vi "SimulatorOscilloscope.vi"() -> ()   [LabVIEW 2014]
uses:
  SimulatorGlobalOscilloscope.vi
panel:
  out "ChkSum Error":bool
  out "Sync Error":bool
  out "Timeout Error":bool
  in  "SimulatorOscilloscope":T1(tab)=enum."Oscilloscope"
  in  "Voltage Reference":dbl caption="V"
  in  "ChkSum":enum16{"ZERO16", "LRC8", "CRC16-CCITT"}(ring)
  in  "Serial Port":T2(ring)
  in  "Baud Rate":u32=9600
  in  "timeout [ms]":u32=10000
  in  "SW":u8
  in  "BTN0":bool
  in  "BTN1":bool
  in  "BTN2":bool
  in  "BTN3":bool
  out "FreqSelect":bool
  out "AmplSelect":bool
  out "ShapeSelect":bool=TRUE
  out "Shape1Index":u8
  out "AmplIndex":u8
  out "FreqIndex":u8
  out "Frequency":string="   0,0Hz"
  out "Amplitude":string="   0,00 V"
  out "Shape":string="Const"
  in  "Number of Packets shown":i16=2
  in  "SEND Button":bool
  in  "Record Length":u16=500
  in  "Sample Rate":u16=10000
  out "Oscilloskop":u8[](graph)
  out "XY Graph":cluster{u32[], dbl[]}(graph)
  in  "Start":bool
  out "Raw Packet":string
  out "Raw":string
  # "Received raw data (in hex)"
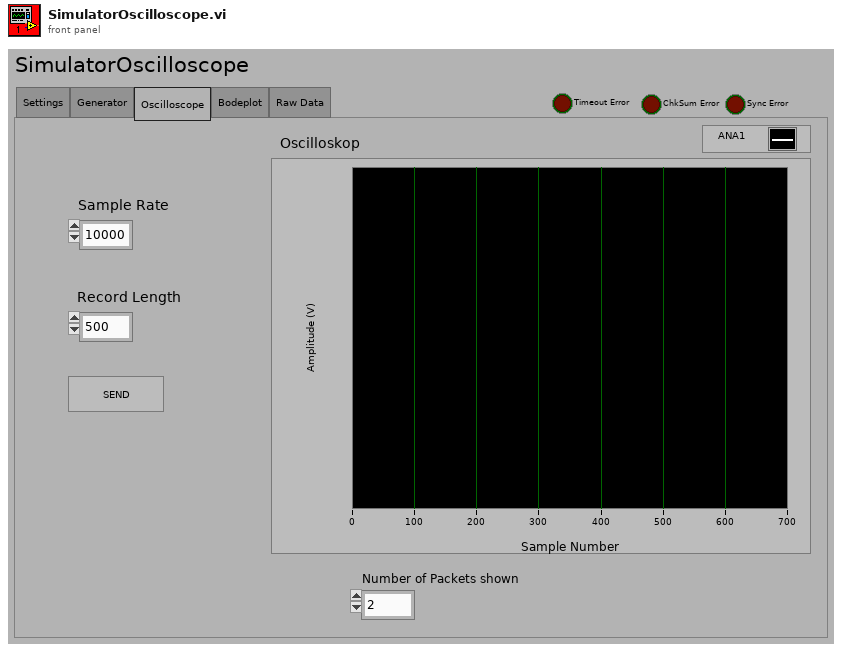
[diagram p1: front panel]
types:
  T1 = enum32{"Settings", "Generator", "Oscilloscope", "Bodeplot", "Raw Data"}
  T2 = enum16{"COM1", "COM2", "COM3", "COM4", "COM5", "COM6", "COM7", "COM8", "COM9", "COM10", "COM11", "COM12", "COM13", "COM14", "COM15", "COM16", "COM17", "COM18", "COM19", "COM20", "COM21", "COM22", "COM23", "COM24", "COM25", "COM26", "COM27", "COM28", "COM29", "COM30"}
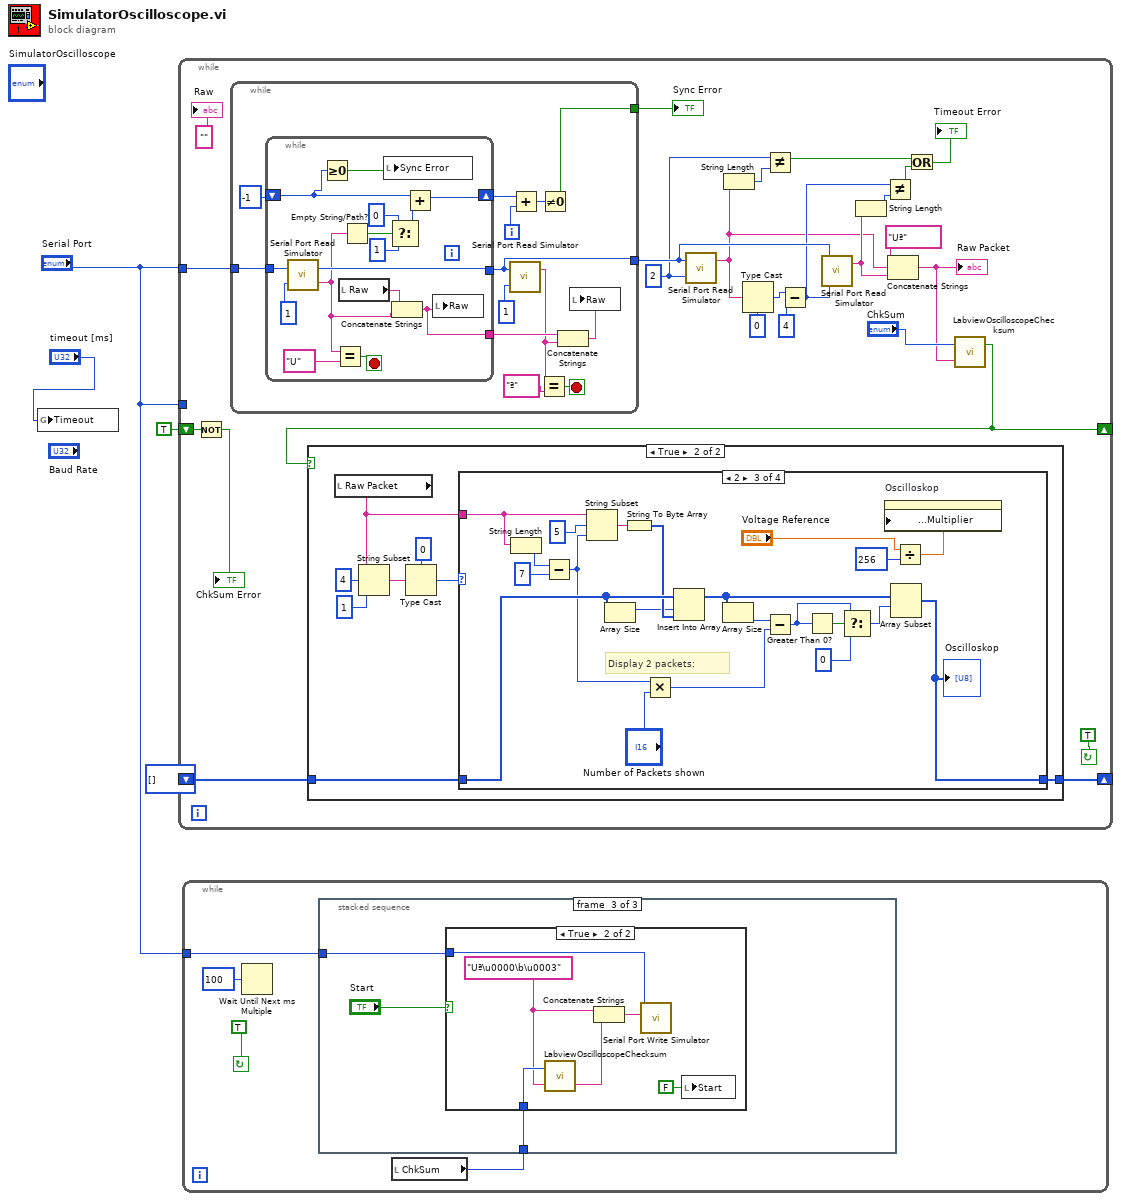
[diagram p0: block diagram]
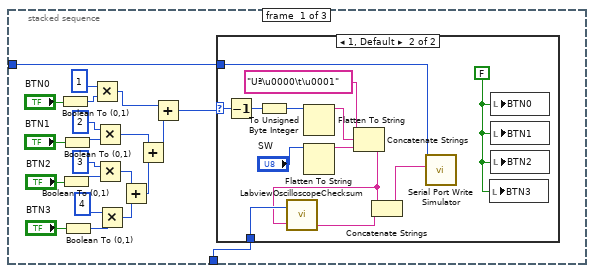
[diagram p2: hidden frame]
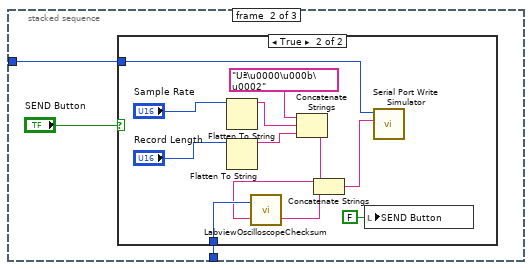
[diagram p4: hidden frame]
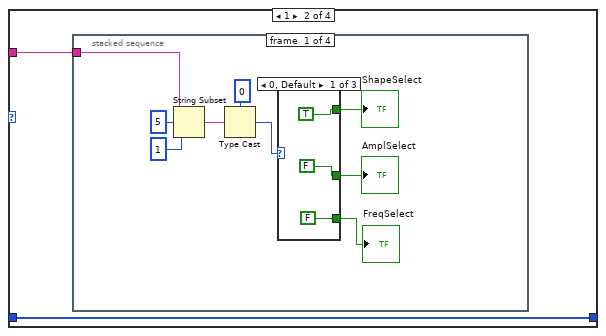
[diagram p9: hidden frame]
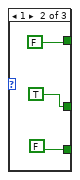
[diagram p10: hidden frame]
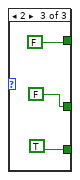
[diagram p11: hidden frame]
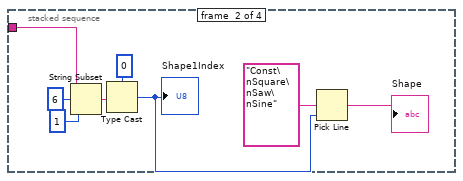
[diagram p12: hidden frame]
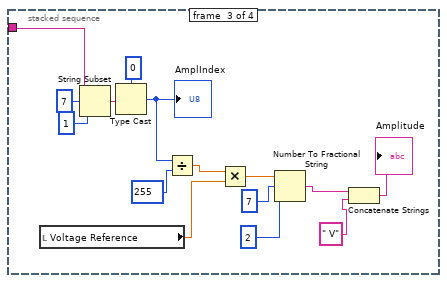
[diagram p13: hidden frame]
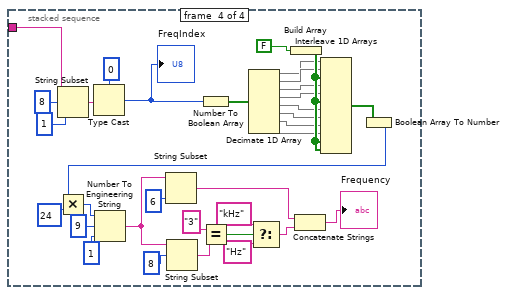
[diagram p14: hidden frame]
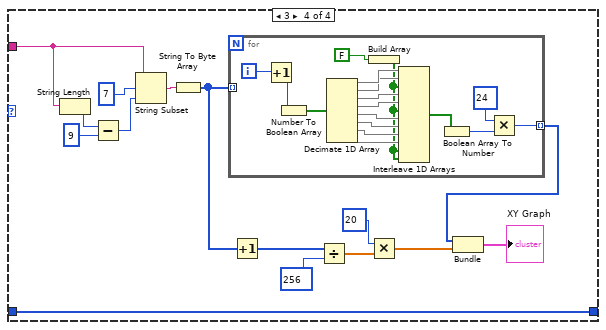
[diagram p15: hidden frame]
diagram:
  n1 = global write "SimulatorGlobalOscilloscope.vi" "Timeout"("timeout [ms]") -> ()
  n2 = while {
    shift-right: [w29] -> _
    shift-left: u8[] [] -> [w28]
    tunnel: "Serial Port" -> [w21]
    shift-right: [w7] -> _
    shift-left: TRUE -> [w6]
    tunnel: "Serial Port" -> [_]
    stop <- TRUE continue-if-true
    w15 = 2
    n3 = Not(x=w6) -> (.not. x?=→"ChkSum Error":bool)
    n4 = while {
      tunnel: w21 -> [w182]
      tunnel: [w177] -> w24
      tunnel: [w178] -> w20
      i -> [w173]
      stop <- w181 stop-if-true
      n5 = while {
        tunnel: w182 -> [w193]
        tunnel: [w193] -> w177
        tunnel: [w183] -> w180
        shift-right: [w185] -> w172
        shift-left: -1 -> [w187]
        stop <- w195 stop-if-true
        n6 = call "Serial Port Read Simulator.vi"("requested byte count"=1, "port number"=w193) -> ("string read"=w184:string)  [unwired: 1 out]
        n7 = Greater Or Equal To 0?(x=w187) -> (x >= 0?=w186:bool)
        n8 = Equal?(x=w184, y="U") -> (x = y?=w195:bool)
        n9 = local read "Raw"() -> (w192:string)
        n10 = Empty String/Path?(string/path=w184) -> (empty?=w188:bool)
        n11 = local write "Sync Error"(w186) -> ()
        n12 = Select(t=0, s=w188, f=1) -> (s? t:f=w189:i32)
        n13 = Concatenate Strings(w192, w184) -> (w183:string)
        n14 = Add(x=w187, y=w189) -> (x+y=w185:i32)
        n15 = local write "Raw"(w183) -> ()
      }
      n16 = call "Serial Port Read Simulator.vi"("requested byte count"=1, "port number"=w177) -> ("string read"=w171:string)  [unwired: 1 out]
      n17 = Add(x=w172, y=w173) -> (x+y=w179:i32)
      n18 = Equal?(x=w171, y="ª") -> (x = y?=w181:bool)
      n19 = Not Equal To 0?(x=w179) -> (x != 0?=w178:bool)
      n20 = Concatenate Strings(w180, w171) -> (w175:string)
      n21 = local write "Raw"(w175) -> ()
    }
    "Sync Error" <- w20
    n22 = call "Serial Port Read Simulator.vi"("requested byte count"=w15, "port number"=w24) -> ("string read"=w11:string)  [unwired: 1 out]
    n23 = String Length(string=w11) -> (length=w18:i32)
    n24 = Type Cast(type=i16 0, x=w11) -> (*(type *) &x=w25:i16)
    n25 = Not Equal?(x=w15, y=w18) -> (x != y?=w16:bool)
    n26 = Subtract(x=w25, y=i16 4) -> (x-y=w14:i16)
    n27 = call "Serial Port Read Simulator.vi"("requested byte count"=w14, "port number"=w24) -> ("string read"=w12:string)  [unwired: 1 out]
    n28 = String Length(string=w12) -> (length=w19:i32)
    n29 = Not Equal?(x=w14, y=w19) -> (x != y?=w17:bool)
    n30 = Concatenate Strings("Uª", w11, w12) -> (w8:string)
    "Raw Packet" <- w8
    n31 = Or(x=w16, y=w17) -> (x .or. y?=→"Timeout Error":bool)
    n32 = call "LabviewOscilloscopeChecksum.vi"("DATA PACKET"=w8, "ChkSumType"="ChkSum") -> ("Checked"=w7:bool)  [unwired: 1 out]
    n33 = case shown="True" w7 {
      tunnel: [w30 w38] -> w29
      tunnel: w28 -> [w30 w37]
      frame False {
      }
      frame True {
        n34 = local read "Raw Packet"() -> (w33:string)
        n35 = String Subset(string=w33, offset (0)=4, length (rest)=1 ("length (rest)")) -> (substring=w36:string)
        n36 = Type Cast(type=u8 0, x=w36) -> (*(type *) &x=w32:u8)
        n37 = case shown="2" w32 {
          tunnel: w33 -> [_ w41 w118 w147]
          tunnel: [w39 w40 w123 w138] -> w38
          tunnel: w37 -> [w39 w40 w131 w138]
          frame 0, Default {
          }
          frame 1 {
            n38 = stacked-sequence {
              tunnel: w41 -> [w48 w63 w78 w112]
              frame #0 {
                n39 = String Subset(string=w48, offset (0)=5, length (rest)=1 ("length (rest)")) -> (substring=w47:string)
                n40 = Type Cast(type=u8 0, x=w47) -> (*(type *) &x=w45:u8)
                n41 = case shown="0, Default" w45 {
                  tunnel: [TRUE FALSE FALSE] -> w44
                  tunnel: [FALSE TRUE FALSE] -> w43
                  tunnel: [FALSE FALSE TRUE] -> w42
                  frame 0, Default {
                  }
                  frame 1 {
                  }
                  frame 2 {
                  }
                }
                "ShapeSelect" <- w44
                "AmplSelect" <- w43
                "FreqSelect" <- w42
              }
              frame #1 {
                n42 = String Subset(string=w63, offset (0)=6, length (rest)=1 ("length (rest)")) -> (substring=w65:string)
                n43 = Type Cast(type=u8 0, x=w65) -> (*(type *) &x=w61:u8)
                "Shape1Index" <- w61
                n44 = Pick Line(multi-line string="Const\nSquare\nSaw\nSine", line index=w61) -> (output string=→"Shape":string)  [unwired: 1 in]
              }
              frame #2 {
                n45 = local read "Voltage Reference"() -> (w68:dbl)
                n46 = String Subset(string=w78, offset (0)=7, length (rest)=1 ("length (rest)")) -> (substring=w81:string)
                n47 = Type Cast(type=u8 0, x=w81) -> (*(type *) &x=w77:u8)
                "AmplIndex" <- w77
                n48 = Divide(x=w77, y=255) -> (x/y=w75:dbl)
                n49 = Multiply(x=w75, y=w68) -> (x*y=w74:dbl)
                n50 = Number To Fractional String(number=w74, width (-)=7, precision (6)=2) -> (F-format string=w71:string)  [unwired: 1 in]
                n51 = Concatenate Strings(w71, " V") -> (→"Amplitude":string)
              }
              frame #3 {
                n52 = String Subset(string=w112, offset (0)=8, length (rest)=1 ("length (rest)")) -> (substring=w114:string)
                n53 = Type Cast(type=u8 0, x=w114) -> (*(type *) &x=w84:u8)
                "FreqIndex" <- w84
                n54 = Number To Boolean Array(number=w84) -> (Boolean array=w86:bool[])
                n55 = Decimate 1D Array(w86) -> (w87:bool[], w93:bool[], w88:bool[], w94:bool[], w89:bool[], w90:bool[], w91:bool[], w95:bool[])
                n56 = Build Array(FALSE) -> (w96:bool[])
                n57 = Interleave 1D Arrays(w87, w93, w96, w88, w94, w96, w89, w90, w91, w95, w96, w96) -> (w92:bool[])
                n58 = Boolean Array To Number(Boolean array=w92) -> (number=w97:u32)
                n59 = Multiply(x=w97, y=24) -> (x*y=w99:u32)
                n60 = Number To Engineering String(2:1, 3:9, 4:w99) -> (0:w104:string)  [unwired: 1 in]
                n61 = String Subset(string=w104, length (rest)=6) -> (substring=w111:string)  [unwired: 1 in]
                n62 = String Subset(string=w104, offset (0)=8) -> (substring=w109:string)  [unwired: 1 in]
                n63 = Equal?(x="3", y=w109) -> (x = y?=w107:bool)
                n64 = Select(t="kHz", s=w107, f="Hz") -> (s? t:f=w110:string)
                n65 = Concatenate Strings(w111, w110) -> (→"Frequency":string)
              }
            }
          }
          frame 2 {
            # "Display 2 packets:"
            n66 = String Length(string=w118) -> (length=w137:i32)
            n67 = Subtract(x=w137, y=7 ("length (rest)")) -> (x-y=w119:i32)
            n68 = String Subset(string=w118, offset (0)=5, length (rest)=w119) -> (substring=w134:string)
            n69 = Array Size(array=w131) -> (size(s)=w129:i32)
            n70 = String To Byte Array(string=w134) -> (unsigned byte array=w130:u8[])
            n71 = Multiply(x=w119, y="Number of Packets shown") -> (x*y=w121:i32)
            n72 = Insert Into Array(array=w131, index=w129, new element=w130) -> (w124:u8[])
            n73 = Array Size(array=w124) -> (size(s)=w126:i32)
            n74 = Subtract(x=w126, y=w121) -> (x-y=w127:i32)
            n75 = Greater Than 0?(x=w127) -> (x > 0?=w128:bool)
            n76 = Select(t=w127, s=w128, f=0) -> (s? t:f=w122:i32)
            n77 = Array Subset(array=w124, index=w122) -> (w123:u8[])  [unwired: 1 in]
            "Oscilloskop" <- w123
            n78 = Divide(x="Voltage Reference", y=u16 256) -> (x/y=w132:dbl)
            n79 = property on="Oscilloskop" class="WFGraph (strict)"("Y Scale.Offset and Multiplier:Multiplier"=w132) -> ()  [unwired: 2 in, 2 out]
          }
          frame 3 {
            n80 = String Length(string=w147) -> (length=w149:i32)
            n81 = Subtract(x=w149, y=9 ("length (rest)")) -> (x-y=w148:i32)
            n82 = String Subset(string=w147, offset (0)=7, length (rest)=w148) -> (substring=w152:string)
            n83 = String To Byte Array(string=w152) -> (unsigned byte array=w143:u8[])
            n84 = for {
              tunnel: [w155] -> w146 mode=indexing
              tunnel: w143 -> [_] mode=indexing
              i -> [w157]
              n85 = Increment(x=w157) -> (x+1=w156:i32)
              n86 = Number To Boolean Array(number=w156) -> (Boolean array=w168:bool[])
              n87 = Decimate 1D Array(w168) -> (w167:bool[], w161:bool[], w166:bool[], w160:bool[], w165:bool[], w164:bool[], w163:bool[], w159:bool[])
              n88 = Build Array(FALSE) -> (w158:bool[])
              n89 = Interleave 1D Arrays(w167, w161, w158, w166, w160, w158, w165, w164, w163, w159, w158, w158) -> (w162:bool[])
              n90 = Boolean Array To Number(Boolean array=w162) -> (number=w154:u32)
              n91 = Multiply(x=24, y=w154) -> (x*y=w155:u32)
            }
            n92 = Increment(x=w143) -> (x+1=w139:u8[])
            n93 = Divide(x=w139, y=256) -> (x/y=w142:dbl[])
            n94 = Multiply(x=20, y=w142) -> (x*y=w140:dbl[])
            n95 = Bundle(w146, w140) -> (→"XY Graph":cluster{u32[], dbl[]})  [unwired: 1 in]
          }
        }
      }
    }
    "Raw" <- ""
  }
  n96 = while {
    tunnel: "Serial Port" -> [w198]
    stop <- TRUE continue-if-true
    n97 = Wait Until Next ms Multiple(millisecond multiple=100) -> ()  [unwired: 1 out]
    n98 = local read "ChkSum"() -> (w197:enum16{"ZERO16", "LRC8", "CRC16-CCITT"})
    n99 = stacked-sequence {
      tunnel: w198 -> [w221 w236 w250]
      tunnel: w197 -> [w220 w235 w249]
      frame #0 {
        n100 = Boolean To (0,1)(Boolean="BTN0") -> (0, 1=w215:i16)
        n101 = Boolean To (0,1)(Boolean="BTN2") -> (0, 1=w211:i16)
        n102 = Boolean To (0,1)(Boolean="BTN1") -> (0, 1=w209:i16)
        n103 = Boolean To (0,1)(Boolean="BTN3") -> (0, 1=w213:i16)
        n104 = Multiply(x=u8 1, y=w215) -> (x*y=w207:i16)
        n105 = Multiply(x=u8 2, y=w209) -> (x*y=w205:i16)
        n106 = Multiply(x=u8 3, y=w211) -> (x*y=w203:i16)
        n107 = Multiply(x=u8 4, y=w213) -> (x*y=w204:i16)
        n108 = Add(x=w203, y=w204) -> (x+y=w202:i16)
        n109 = Add(x=w205, y=w202) -> (x+y=w206:i16)
        n110 = Add(x=w207, y=w206) -> (x+y=w201:i16)
        n111 = case shown="1, Default" w201 {
          selector: w201 -> [_ w230]
          tunnel: w221 -> [_ w224]
          tunnel: w220 -> [_ w228]
          frame 0 {
          }
          frame 1, Default {
            w231 = FALSE
            n112 = Decrement(x=w230) -> (x-1=w225:i16)
            n113 = To Unsigned Byte Integer(number=w225) -> (unsigned 8bit integer=w222:u8)
            n114 = Flatten To String(anything=w222) -> (data string=w229:string)  [unwired: 3 in, 2 out]
            n115 = Flatten To String(anything="SW") -> (data string=w232:string)  [unwired: 3 in, 2 out]
            n116 = Concatenate Strings("Uª\u0000\t\u0001", w229, w232) -> (w226:string)
            n117 = call "LabviewOscilloscopeChecksum.vi"("DATA PACKET"=w226, "ChkSumType"=w228) -> ("ChkSum"=w227:string)  [unwired: 1 out]
            n118 = Concatenate Strings(w226, w227) -> (w223:string)
            n119 = call "Serial Port Write Simulator.vi"("Port"=w224, "String"=w223) -> ()  [unwired: 6 in]
            n120 = local write "BTN3"(w231) -> ()
            n121 = local write "BTN0"(w231) -> ()
            n122 = local write "BTN1"(w231) -> ()
            n123 = local write "BTN2"(w231) -> ()
          }
        }
      }
      frame #1 {
        n124 = case shown="True" "SEND Button" {
          tunnel: w236 -> [_ w242]
          tunnel: w235 -> [_ w241]
          frame False {
          }
          frame True {
            n125 = Flatten To String(anything="Sample Rate") -> (data string=w247:string)  [unwired: 3 in, 2 out]
            n126 = Flatten To String(anything="Record Length") -> (data string=w246:string)  [unwired: 3 in, 2 out]
            n127 = Concatenate Strings("Uª\u0000\u000b\u0002", w247, w246) -> (w240:string)
            n128 = call "LabviewOscilloscopeChecksum.vi"("DATA PACKET"=w240, "ChkSumType"=w241) -> ("ChkSum"=w239:string)  [unwired: 1 out]
            n129 = Concatenate Strings(w240, w239) -> (w238:string)
            n130 = local write "SEND Button"(FALSE) -> ()
            n131 = call "Serial Port Write Simulator.vi"("Port"=w242, "String"=w238) -> ()  [unwired: 6 in]
          }
        }
      }
      frame #2 {
        n132 = case shown="True" "Start" {
          tunnel: w250 -> [_ w256]
          tunnel: w249 -> [_ w255]
          frame False {
          }
          frame True {
            w253 = "Uª\u0000\b\u0003"
            n133 = call "LabviewOscilloscopeChecksum.vi"("DATA PACKET"=w253, "ChkSumType"=w255) -> ("ChkSum"=w252:string)  [unwired: 1 out]
            n134 = Concatenate Strings(w253, w252) -> (w254:string)
            n135 = call "Serial Port Write Simulator.vi"("Port"=w256, "String"=w254) -> ()  [unwired: 6 in]
            n136 = local write "Start"(FALSE) -> ()
          }
        }
      }
    }
  }
